vi "set tag writer or reader.vi"(7 "module GUID":string, 8 "error in":errorcluster, 9 "channel":refnum<class "TBM channel.lvclass">, 10 "tag descriptor":refnum<class "tag descriptor.lvclass">, 11 "engine configuration in":refnum<class "engine configuration.lvclass">) -> (0 "error out":errorcluster, 3 "engine configuration out":refnum<class "engine configuration.lvclass">)   [LabVIEW 2014, in "engine configuration.lvclass"]
uses:
  engine configuration.lvclass
  <vilib>/NI/Tag Bus/tag/tag descriptor.lvclass
  <vilib>/NI/Tag Bus Module Framework/channel/TBM channel.lvclass
  <vilib>/NI/Tag Bus/tag/tag descriptor.lvclass/tag descriptor.ctl
  <vilib>/NI/Tag Bus Module Framework/channel/TBM channel.lvclass/TBM channel.ctl
  engine configuration.lvclass/engine configuration.ctl
  <vilib>/NI/Tag Bus Module Framework/channel/Read channel classification.vi
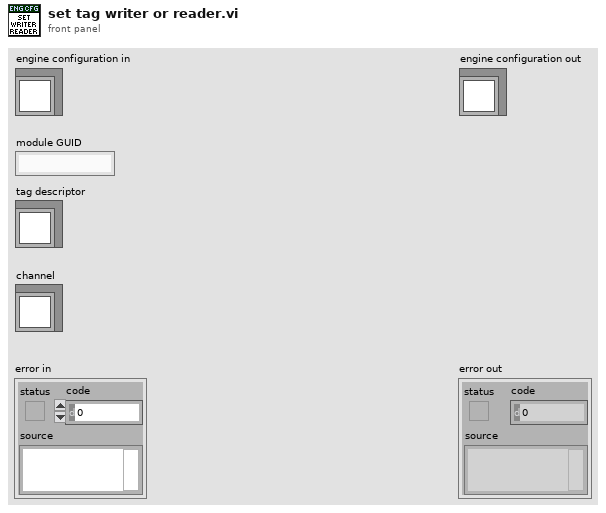
[diagram p1: front panel]
types:
  T1 = typedef "TBM channel.lvclass/channel classification.ctl" = enum16{"input data", "output data", "processing parameter", "processing result"}
  T2 = typedef "engine configuration.lvclass/module channel pairings.ctl" = cluster{"modules":string[], "channels":string[]}
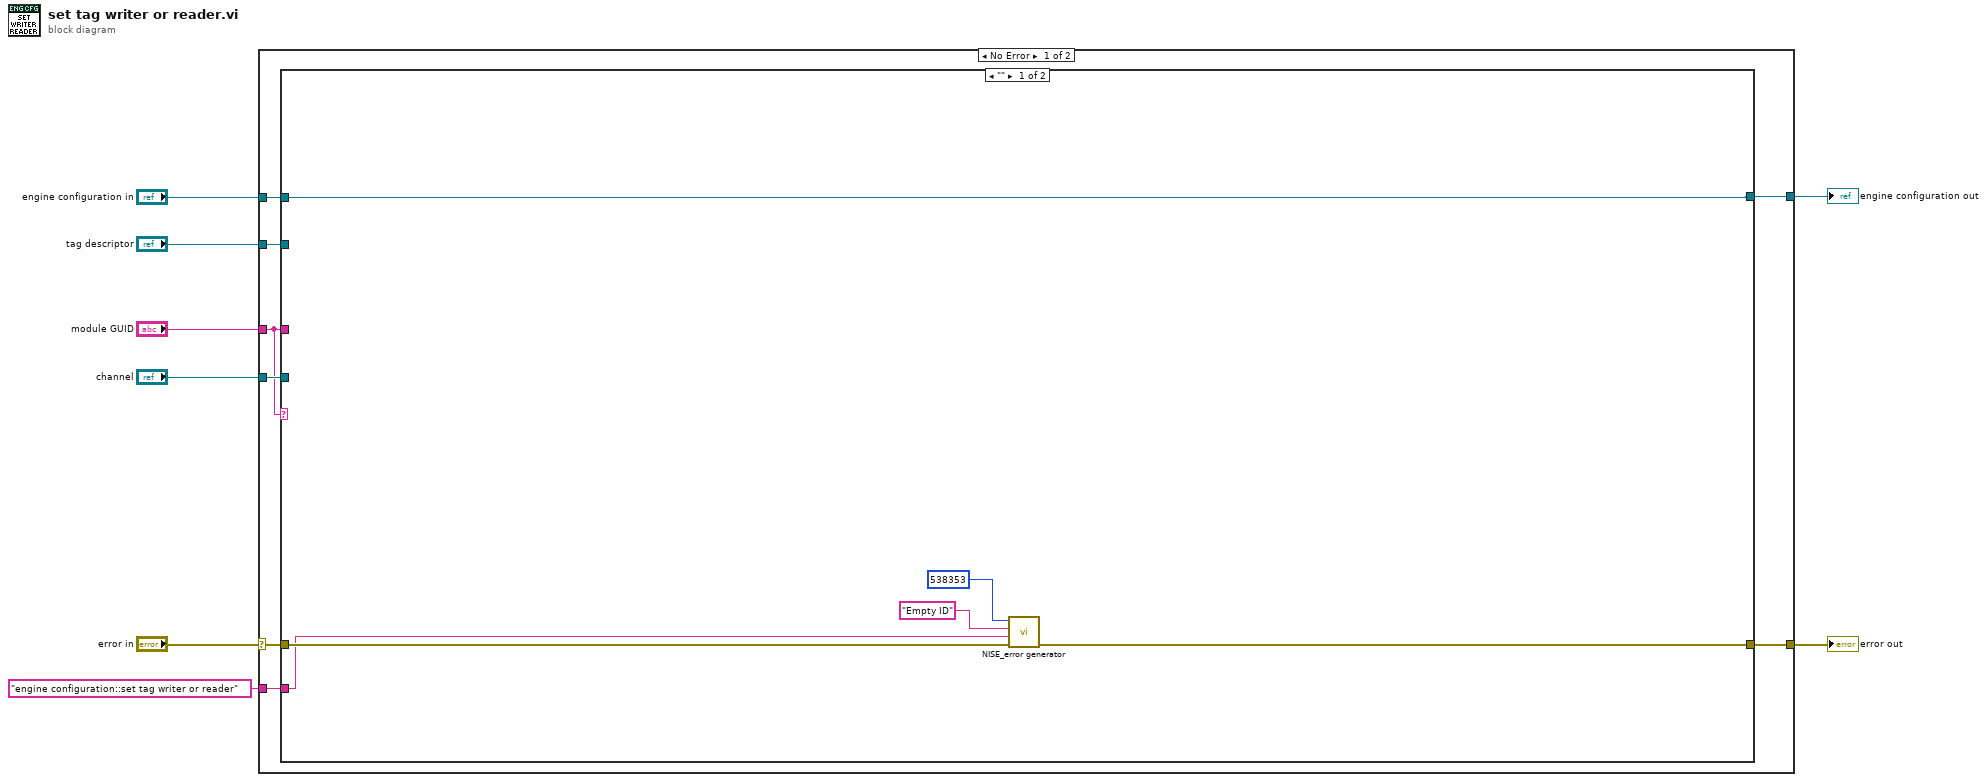
[diagram p0: block diagram]
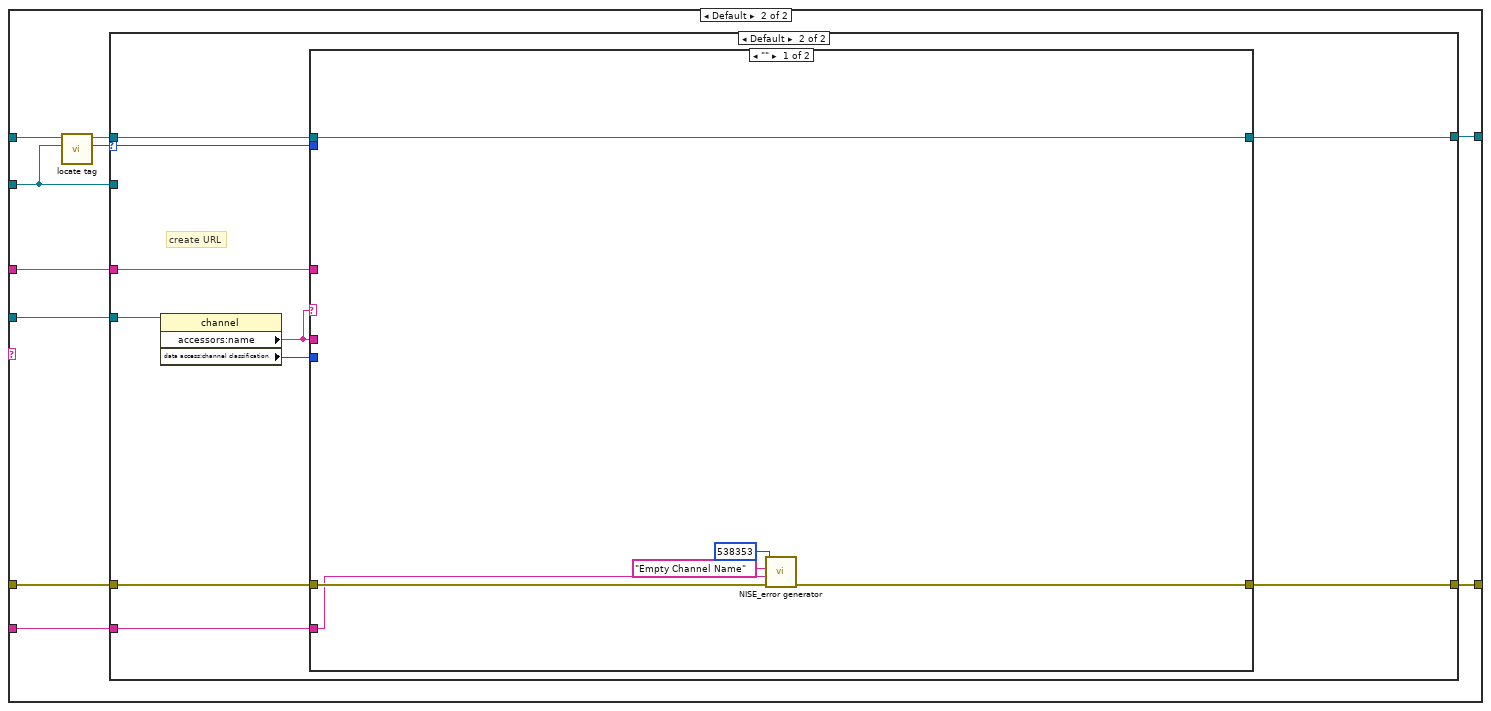
[diagram p2: hidden frame]
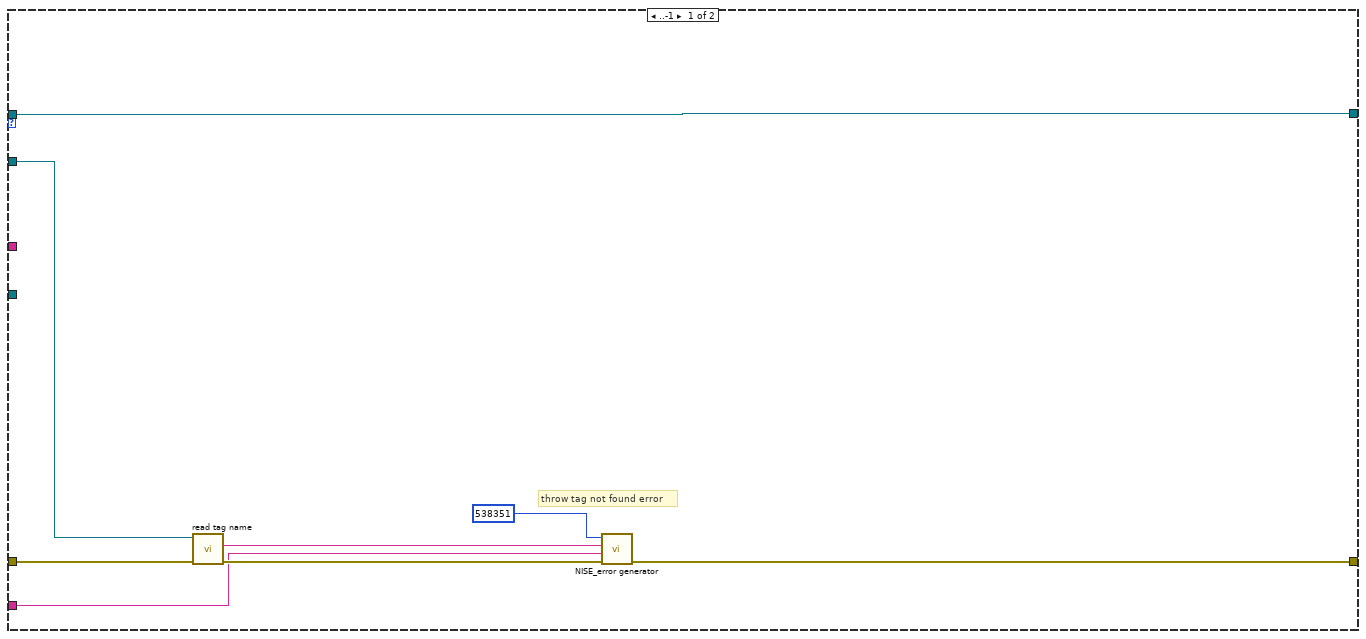
[diagram p3: hidden frame]
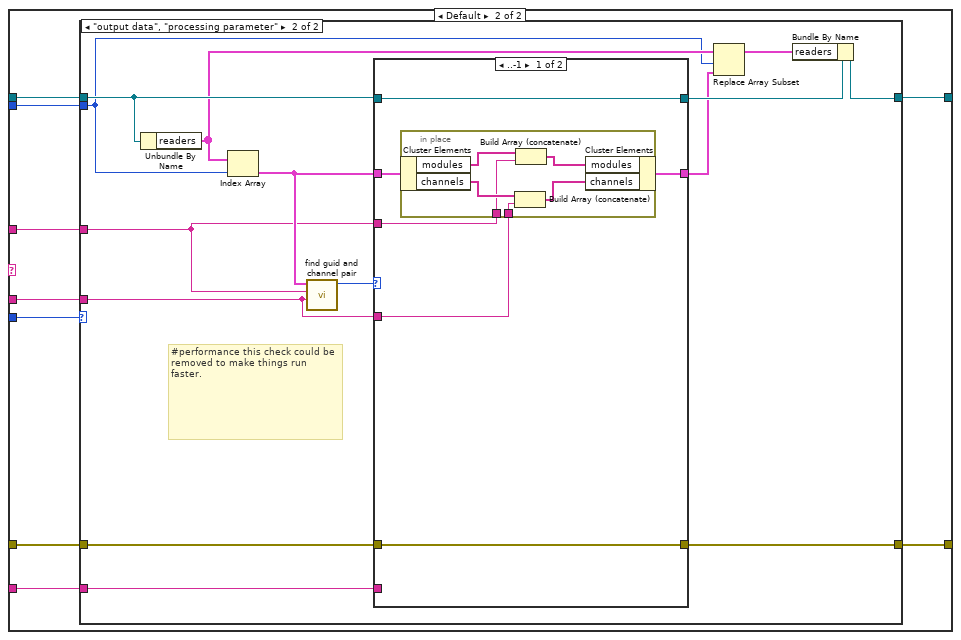
[diagram p4: hidden frame]
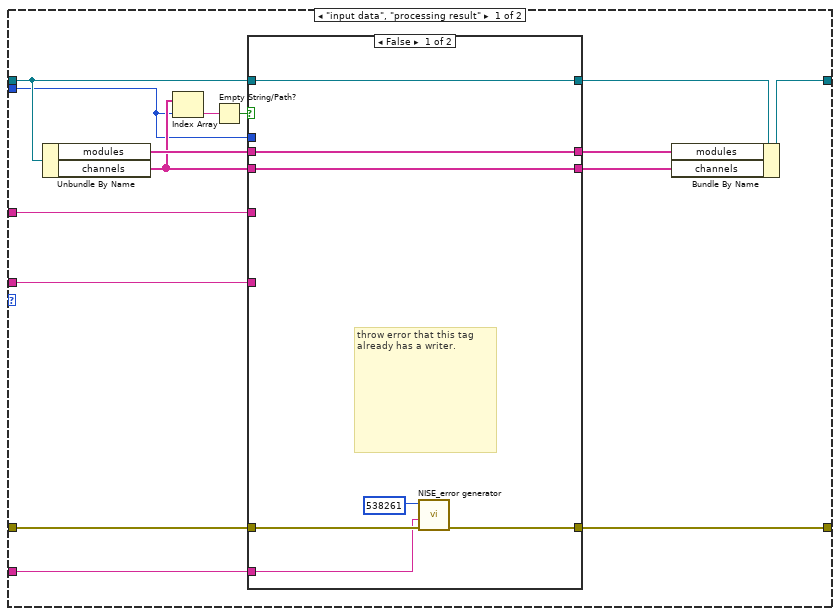
[diagram p5: hidden frame]
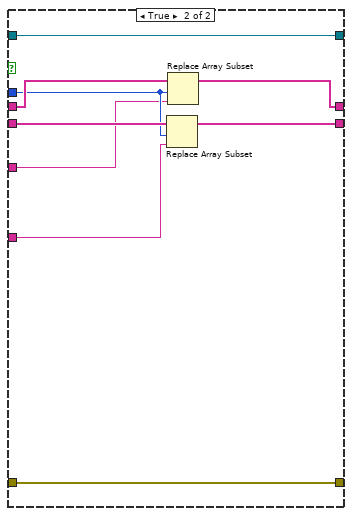
[diagram p6: hidden frame]
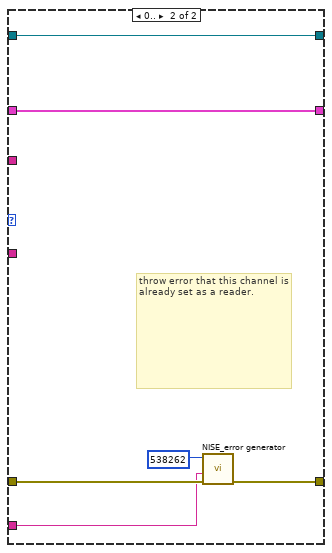
[diagram p7: hidden frame]
diagram:
  n1 = case shown="No Error" "error in" {
    selector: "error in" -> [w14 w130]
    tunnel: [w13 w130] -> w7
    tunnel: [w12 w129] -> w5
    tunnel: "engine configuration in" -> [w16 w129]
    tunnel: "tag descriptor" -> [w11 _]
    tunnel: "module GUID" -> [w9 _]
    tunnel: "channel" -> [w15 _]
    tunnel: "engine configuration::set tag writer or reader" ("source") -> [w10 _]
    frame No Error {
      n2 = case shown="\"\"" w9 {
        tunnel: w16 -> [w22 w32]
        tunnel: w15 -> [_ w30]
        tunnel: w9 -> [_ w29]
        tunnel: w14 -> [w21 w28]
        tunnel: [w20 w26] -> w13
        tunnel: [w22 w25] -> w12
        tunnel: w11 -> [_ w24]
        tunnel: w10 -> [w19 w23]
        frame "" {
          n3 = call <vilib>:"NISE_error generator.vi"("error in"=w21, "source"=w19, "append error message"="Empty ID", "error code (0)"=538353) -> ("error out"=w20:errorcluster)  [unwired: 5 in]
        }
        frame Default {
          n4 = call "locate tag.vi"("tag descriptor"=w24, "engine configuration in"=w32) -> ("index"=w27:i32, "engine configuration out"=w31:refnum<class "engine configuration.lvclass">)  [unwired: 8 in]
          n5 = case shown="Default" w27 {
            selector: w27 -> [_ w47]
            tunnel: w31 -> [w40 w46]
            tunnel: w30 -> [_ w50]
            tunnel: w29 -> [_ w42]
            tunnel: w28 -> [w36 w48]
            tunnel: [w38 w45] -> w26
            tunnel: [w40 w44] -> w25
            tunnel: w24 -> [w37 _]
            tunnel: w23 -> [w33 w43]
            frame ..-1 {
              # "throw tag not found error"
              n6 = call <vilib>:"read tag name.vi"("error in"=w36, "system tag in"=w37) -> ("error out"=w35:errorcluster, "name"=w34:string)  [unwired: 7 in, 1 out]
              n7 = call <vilib>:"NISE_error generator.vi"("error in"=w35, "source"=w33, "append error message"=w34, "error code (0)"=538351) -> ("error out"=w38:errorcluster)  [unwired: 5 in]
            }
            frame Default {
              # "create URL"
              n8 = property class="channel"(reference=w50) -> ("accessors:name"=w41:string, "data access:channel classification"=w49:T1)  [unwired: 1 in, 2 out]
              n9 = case shown="\"\"" w41 {
                tunnel: w49 -> [_ w65]
                tunnel: w48 -> [w55 w64]
                tunnel: w47 -> [_ w63]
                tunnel: w46 -> [w56 w62]
                tunnel: [w54 w61] -> w45
                tunnel: [w56 w60] -> w44
                tunnel: w43 -> [w53 w59]
                tunnel: w41 -> [_ w58]
                tunnel: w42 -> [_ w57]
                frame "" {
                  n10 = call <vilib>:"NISE_error generator.vi"("error in"=w55, "source"=w53, "append error message"="Empty Channel Name", "error code (0)"=538353) -> ("error out"=w54:errorcluster)  [unwired: 5 in]
                }
                frame Default {
                  n11 = case shown="\"output data\", \"processing parameter\"" w65 {
                    tunnel: w64 -> [w80 w109]
                    tunnel: w63 -> [w68 w100]
                    tunnel: w62 -> [w76 w106]
                    tunnel: [w75 w104] -> w60
                    tunnel: [w78 w108] -> w61
                    tunnel: w59 -> [w77 w107]
                    tunnel: w58 -> [w66 w98]
                    tunnel: w57 -> [w67 w97]
                    frame "input data", "processing result" {
                      n12 = Unbundle By Name(w76) -> ("modules"=w72:string[], "channels"=w70:string[])
                      n13 = Index Array(array=w70, index=w68) -> (element=w74:string)
                      n14 = Empty String/Path?(string/path=w74) -> (empty?=w73:bool)
                      n15 = case shown="False" w73 {
                        tunnel: w80 -> [w85 w96]
                        tunnel: [w84 w96] -> w78
                        tunnel: w76 -> [w87 w95]
                        tunnel: [w87 w95] -> w79
                        tunnel: w77 -> [w83 _]
                        tunnel: w72 -> [w82 w91]
                        tunnel: [w82 w92] -> w71
                        tunnel: w70 -> [w81 w94]
                        tunnel: [w81 w93] -> w69
                        tunnel: w68 -> [_ w90]
                        tunnel: w67 -> [_ w89]
                        tunnel: w66 -> [_ w88]
                        frame False {
                          # "throw error that this tag already has a writer."
                          n16 = call <vilib>:"NISE_error generator.vi"("error in"=w85, "source"=w83, "error code (0)"=538261) -> ("error out"=w84:errorcluster)  [unwired: 6 in]
                        }
                        frame True {
                          n17 = Replace Array Subset(array=w94, new element=w88, index=w90) -> (w93:string[])
                          n18 = Replace Array Subset(array=w91, new element=w89, index=w90) -> (w92:string[])
                        }
                      }
                      n19 = Bundle By Name(cluster=w79, "modules"=w71, "channels"=w69) -> (w75:refnum<class "engine configuration.lvclass">)
                    }
                    frame "output data", "processing parameter" {
                      # "#performance this check could be removed to make things run faster."
                      n20 = Unbundle By Name(w106) -> ("readers"=w102:T2[])
                      n21 = Index Array(array=w102, index=w100) -> (element=w103:T2)
                      n22 = call "find guid and channel pair.vi"("channel name"=w98, "Module GUID"=w97, "listing"=w103) -> ("index"=w105:i32)  [unwired: 8 in]
                      n23 = case shown="..-1" w105 {
                        tunnel: w106 -> [w116 w128]
                        tunnel: [w116 w128] -> w110
                        tunnel: w109 -> [w115 w126]
                        tunnel: [w115 w125] -> w108
                        tunnel: w107 -> [_ w124]
                        tunnel: w103 -> [w114 w123]
                        tunnel: [w113 w123] -> w99
                        tunnel: w98 -> [w112 _]
                        tunnel: w97 -> [w111 _]
                        frame ..-1 {
                          n24 = in-place {
                            in-place-border: w112 -> [w118]
                            in-place-border: w111 -> [w117]
                            n25 = in-place-cluster #1(w114) -> ("modules"=w122:string[], "channels"=w120:string[])
                            n26 = Build Array (concatenate)(w120, w118) -> (w119:string[])
                            n27 = Build Array (concatenate)(w122, w117) -> (w121:string[])
                            n28 = in-place-cluster #1("modules"=w121, "channels"=w119) -> (w113:T2)
                          }
                        }
                        frame 0.. {
                          # "throw error that this channel is already set as a reader."
                          n29 = call <vilib>:"NISE_error generator.vi"("error in"=w126, "source"=w124, "error code (0)"=538262) -> ("error out"=w125:errorcluster)  [unwired: 6 in]
                        }
                      }
                      n30 = Replace Array Subset(array=w102, new element=w99, index=w100) -> (w101:T2[])
                      n31 = Bundle By Name(cluster=w110, "readers"=w101) -> (w104:refnum<class "engine configuration.lvclass">)
                    }
                  }
                }
              }
            }
          }
        }
      }
    }
    frame Error {
    }
  }
  "error out" <- w7
  "engine configuration out" <- w5
